vi "Remove Outliers (multiple).vi"(8 "error in (no error)":errorcluster, 9 "Y Lower":dbl, 10 "Y Upper":dbl, 11 "XY-data":cluster{"X-array":dbl[], "Y-array":dbl[]}[](array[cluster])) -> (0 "error out":errorcluster, 3 "XY-data out":cluster{"X-array":dbl[], "Y-array":dbl[]}[](array[cluster]) {"Y-array" format="%.2p"; "X-array" format="%.2p"})   [LabVIEW 2019, in "xy_utilities.lvlib"]
doc: "Remove outliers from the y array of <b>XY-data</b> between <b>Y Upper</b> and <b>Y Lower</b> limits.\n\nWire data to the data input to determine the polymorphic instance to use or manually select the instance."
uses:
  xy_utilities.lvlib
  <vilib>/Analysis/6fits.llb/Remove Outliers.vi
  <vilib>/Analysis/6fits.llb/Remove Outliers (Range).vi
  <vilib>/Utility/error.llb/Error Cluster From Error Code.vi
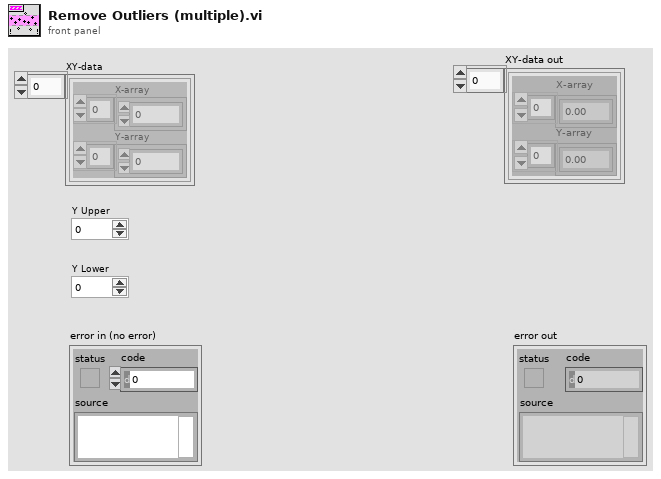
[diagram p1: front panel]
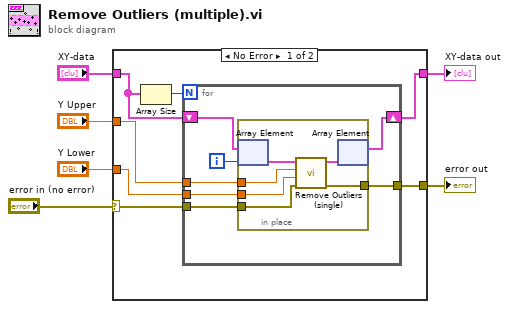
[diagram p0: block diagram]
diagram:
  n1 = case shown="No Error" "error in (no error)" {
    selector: "error in (no error)" -> [w12 w27]
    tunnel: [w13 w27] -> w1
    tunnel: "Y Lower" -> [w11 _]
    tunnel: "Y Upper" -> [w10 _]
    tunnel: "XY-data" -> [w7 w28]
    tunnel: [w9 w28] -> w2
    frame No Error {
      n2 = Array Size(array=w7) -> (size(s)=w8:i32)
      n3 = for {
        N: w8 -> [_]
        tunnel: w11 -> [w19]
        tunnel: w10 -> [w20]
        tunnel: w12 -> [w18]
        tunnel: [w17] -> w13
        shift-right: [w14] -> w9
        shift-left: w7 -> [w16]
        i -> [w15]
        n4 = in-place {
          in-place-border: w20 -> [w26]
          in-place-border: w19 -> [w25]
          in-place-border: w18 -> [w24]
          in-place-border: [w23] -> w17
          n5 = in-place-array #1(w16, w15) -> (w22:cluster{"X-array":dbl[], "Y-array":dbl[]})
          n6 = call "Remove Outliers (single).vi"("error in (no error)"=w24, "Y Lower"=w25, "Y Upper"=w26, "XY-data"=w22) -> ("error out"=w23:errorcluster, "XY-data out"=w21:cluster{"X-array":dbl[], "Y-array":dbl[]})  [unwired: 6 in]
          n7 = in-place-array #1(w21) -> (w14:cluster{"X-array":dbl[], "Y-array":dbl[]}[])  [unwired: 1 out]
        }
      }
    }
    frame Error {
    }
  }
  "error out" <- w1
  "XY-data out" <- w2
